vi "LCD.vi"(6 "String":string, 7 "Direccion":u8 format="%x", 8 "error in (no error)":errorcluster, 9 "Fila":u8, 10 "Columna":u8, 11 "VISA resource name":refnum<visa-resource-name>) -> (0 "error out":errorcluster, 2 "respuesta":string, 3 "VISA resource name out":refnum<visa-resource-name>)   [LabVIEW 2026]
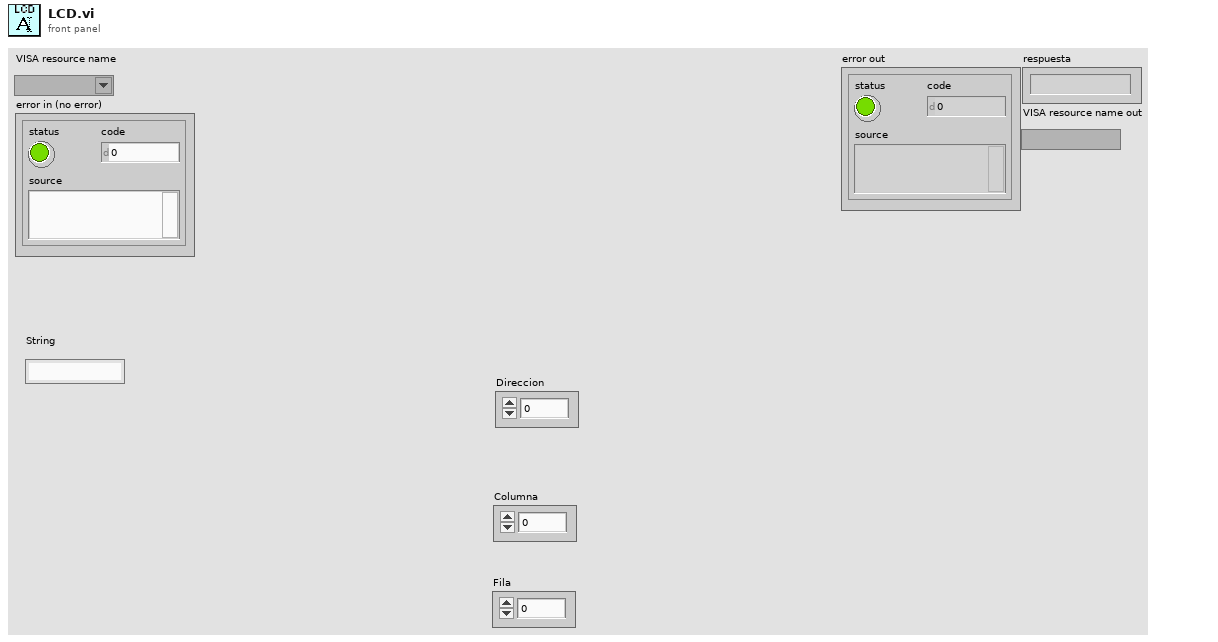
[diagram p1: front panel]
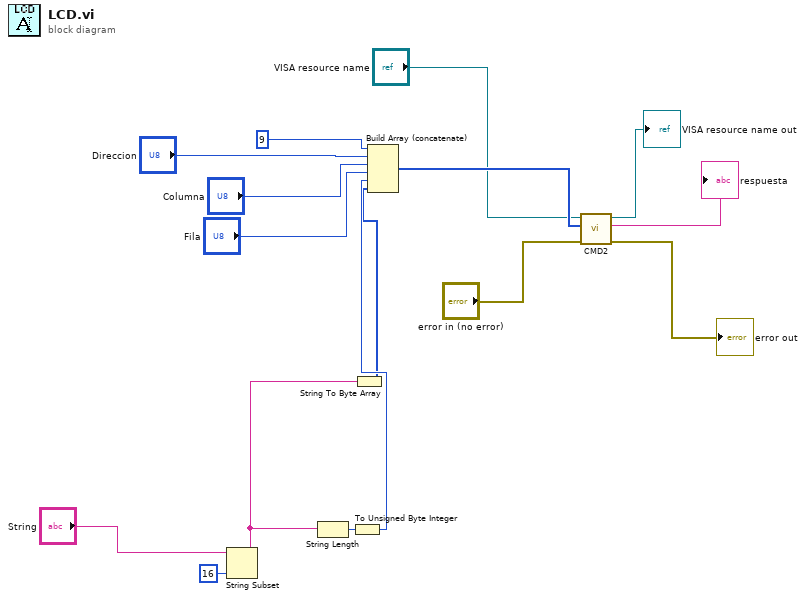
[diagram p0: block diagram]
diagram:
  n1 = String Subset(string="String", length (rest)=16 ("length (rest)")) -> (substring=w6:string)  [unwired: 1 in]
  n2 = String Length(string=w6) -> (length=w3:i32)
  n3 = To Unsigned Byte Integer(number=w3) -> (unsigned 8bit integer=w2:u8)
  n4 = String To Byte Array(string=w6) -> (unsigned byte array=w1:u8[])
  n5 = Build Array (concatenate)(u8 9, "Direccion", "Columna", "Fila", w2, w1) -> (w15:u8[])
  n6 = call "CMD2.vi"("error in (no error)"="error in (no error)", "Comando"=w15, "VISA resource name"="VISA resource name") -> ("error out"=→"error out":errorcluster, "respuesta"=→"respuesta":string, "VISA resource name out"=→"VISA resource name out":refnum<visa-resource-name>)  [unwired: 6 in]
